vi "eDyno CAN Pack Signals.vi"(0 "Fault Injection":T5={"Imbalance ON"=FALSE, "Imbalance (g)"=0.5, "Misalignment ON"=FALSE, "Misalignment (g)"=0.2, "Bearing BPFO ON"=FALSE, "Bearing Impact (g)"=2.0, "Motor Ripple ON"=FALSE, "Torque Ripple (g)"=0.3, "PWM Noise ON"=FALSE, "PWM Level (g)"=0.05}, 5 "Speed Profile":T4={"Run-up Enabled"=FALSE, "Constant Speed (rpm)"=3000.0, "Run-up Start (rpm)"=500.0, "Run-up End (rpm)"=4500.0, "Run-up Duration (s)"=30.0}, 7 "Sim Config":T3={"Sample Rate (Hz)"=51200.0, "Ref Speed (rpm)"=3000.0, "Baseline 1x (g)"=0.02, "Noise Floor (g rms)"=0.01, "BPFO Order"=3.57, "Resonance (Hz)"=3500.0, "Decay (ms)"=0.8, "Pole Pairs"=4.0, "PWM Carrier (Hz)"=16000.0}, 9 "Fault Frequencies (Hz)":T2={"1x Shaft"=50.0, "2x Misalign"=100.0, "BPFO"=178.5, "Torque Ripple"=1200.0, "PWM Carrier"=16000.0}, 11 "Status":T1) -> (4 "Signal Values":dbl[](array[numeric]), 6 "Signal List":string[](array[string]), 8 "Active Fault Id":dbl)   [LabVIEW 2026]
doc: "PURPOSE\nConverts the eDyno simulator state into the 58 signal values of eDyno_NVH_PoC.dbc (v0.5) for an NI-XNET Signal Output Single-point session. Called once per CAN loop iteration.\n\nHOW TO USE\n1) Call it once before the loop and wire Signal List into XNET Create Session (Generic), mode Signal Output Single-point. Signal List is the single source of truth for the order of Signal Values.\n2) In the loop, wire Signal Values into XNET Write (Signal Single-point).\n\nINPUTS\n- Fault Injection, Speed Profile, Sim Config, Fault Frequencies (Hz): the simulator clusters, copied straight into the matching CAN signals.\n- Status: Speed Act (rpm) = shaft speed; Torque (Nm) = motor load torque (drives the MCU model); Block Counter = AO block index; Alive Counter = CAN loop iteration. Test Step and Seq State are no longer sent.\n\nDERIVED SIGNALS (one comment each on the block diagram)\n- Mode: 2 = run-up, 1 = constant speed.\n- AtSpeed: 1 when |Speed Act - target| < 1 rpm (target = Run-up End or Constant Speed).\n- ON flags: boolean -> 1/0.\n- ActiveId: 0 = none, 1..5 = the single fault that is on (Imbalance, Misalignment, BPFO, Torque ripple, PWM), 6 = more than one.\n- Alive counters: Alive Counter mod 16.\n- MCU_Status: computed by eDyno MCU Model.vi from speed and load torque.\n\nCHANGING THE DATABASE\nEvery DBC change must be mirrored here (signal list + values, same order). Check with src/CAN/_aixml/XNET Signal Probe.vi. FlexLogger 2026 Q3 does not decode DBCs with VAL_ value tables."
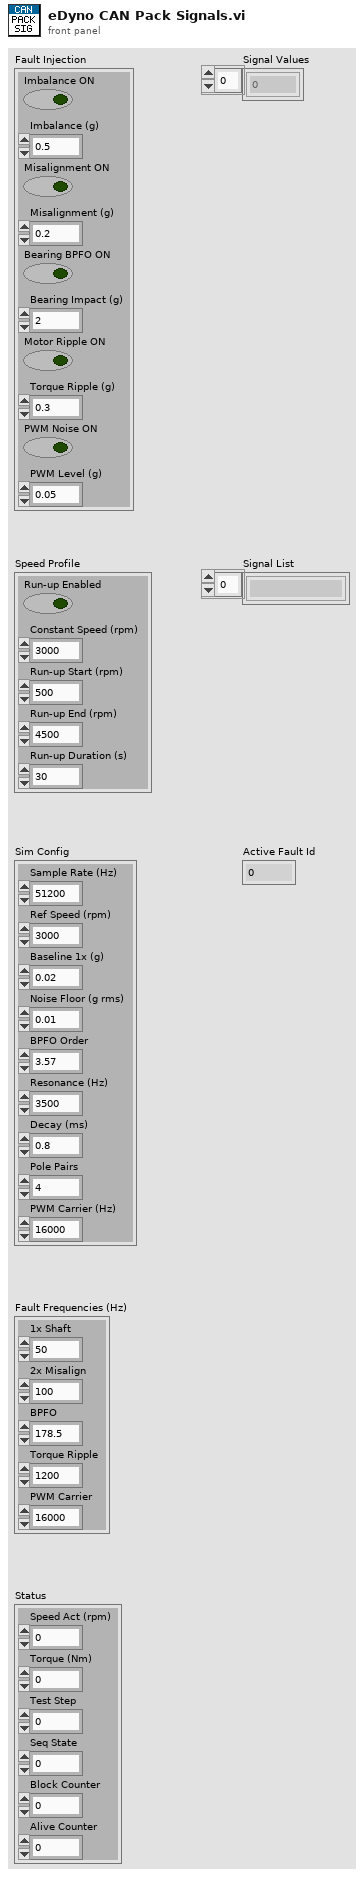
[diagram p1: front panel]
types:
  T1 = cluster{"Speed Act (rpm)":dbl, "Torque (Nm)":dbl, "Test Step":dbl, "Seq State":dbl, "Block Counter":dbl, "Alive Counter":dbl}
  T2 = cluster{"1x Shaft":dbl, "2x Misalign":dbl, "BPFO":dbl, "Torque Ripple":dbl, "PWM Carrier":dbl}
  T3 = cluster{"Sample Rate (Hz)":dbl, "Ref Speed (rpm)":dbl, "Baseline 1x (g)":dbl, "Noise Floor (g rms)":dbl, "BPFO Order":dbl, "Resonance (Hz)":dbl, "Decay (ms)":dbl, "Pole Pairs":dbl, "PWM Carrier (Hz)":dbl}
  T4 = cluster{"Run-up Enabled":bool, "Constant Speed (rpm)":dbl, "Run-up Start (rpm)":dbl, "Run-up End (rpm)":dbl, "Run-up Duration (s)":dbl}
  T5 = cluster{"Imbalance ON":bool, "Imbalance (g)":dbl, "Misalignment ON":bool, "Misalignment (g)":dbl, "Bearing BPFO ON":bool, "Bearing Impact (g)":dbl, "Motor Ripple ON":bool, "Torque Ripple (g)":dbl, "PWM Noise ON":bool, "PWM Level (g)":dbl}
  T6 = cluster{"Motor Speed (rpm)":dbl, "Torque (Nm)":dbl, "Phase Current RMS (A)":dbl, "DC Voltage (V)":dbl, "DC Current (A)":dbl, "Electrical Power (W)":dbl, "Winding Temp (degC)":dbl, "Controller Temp (degC)":dbl}
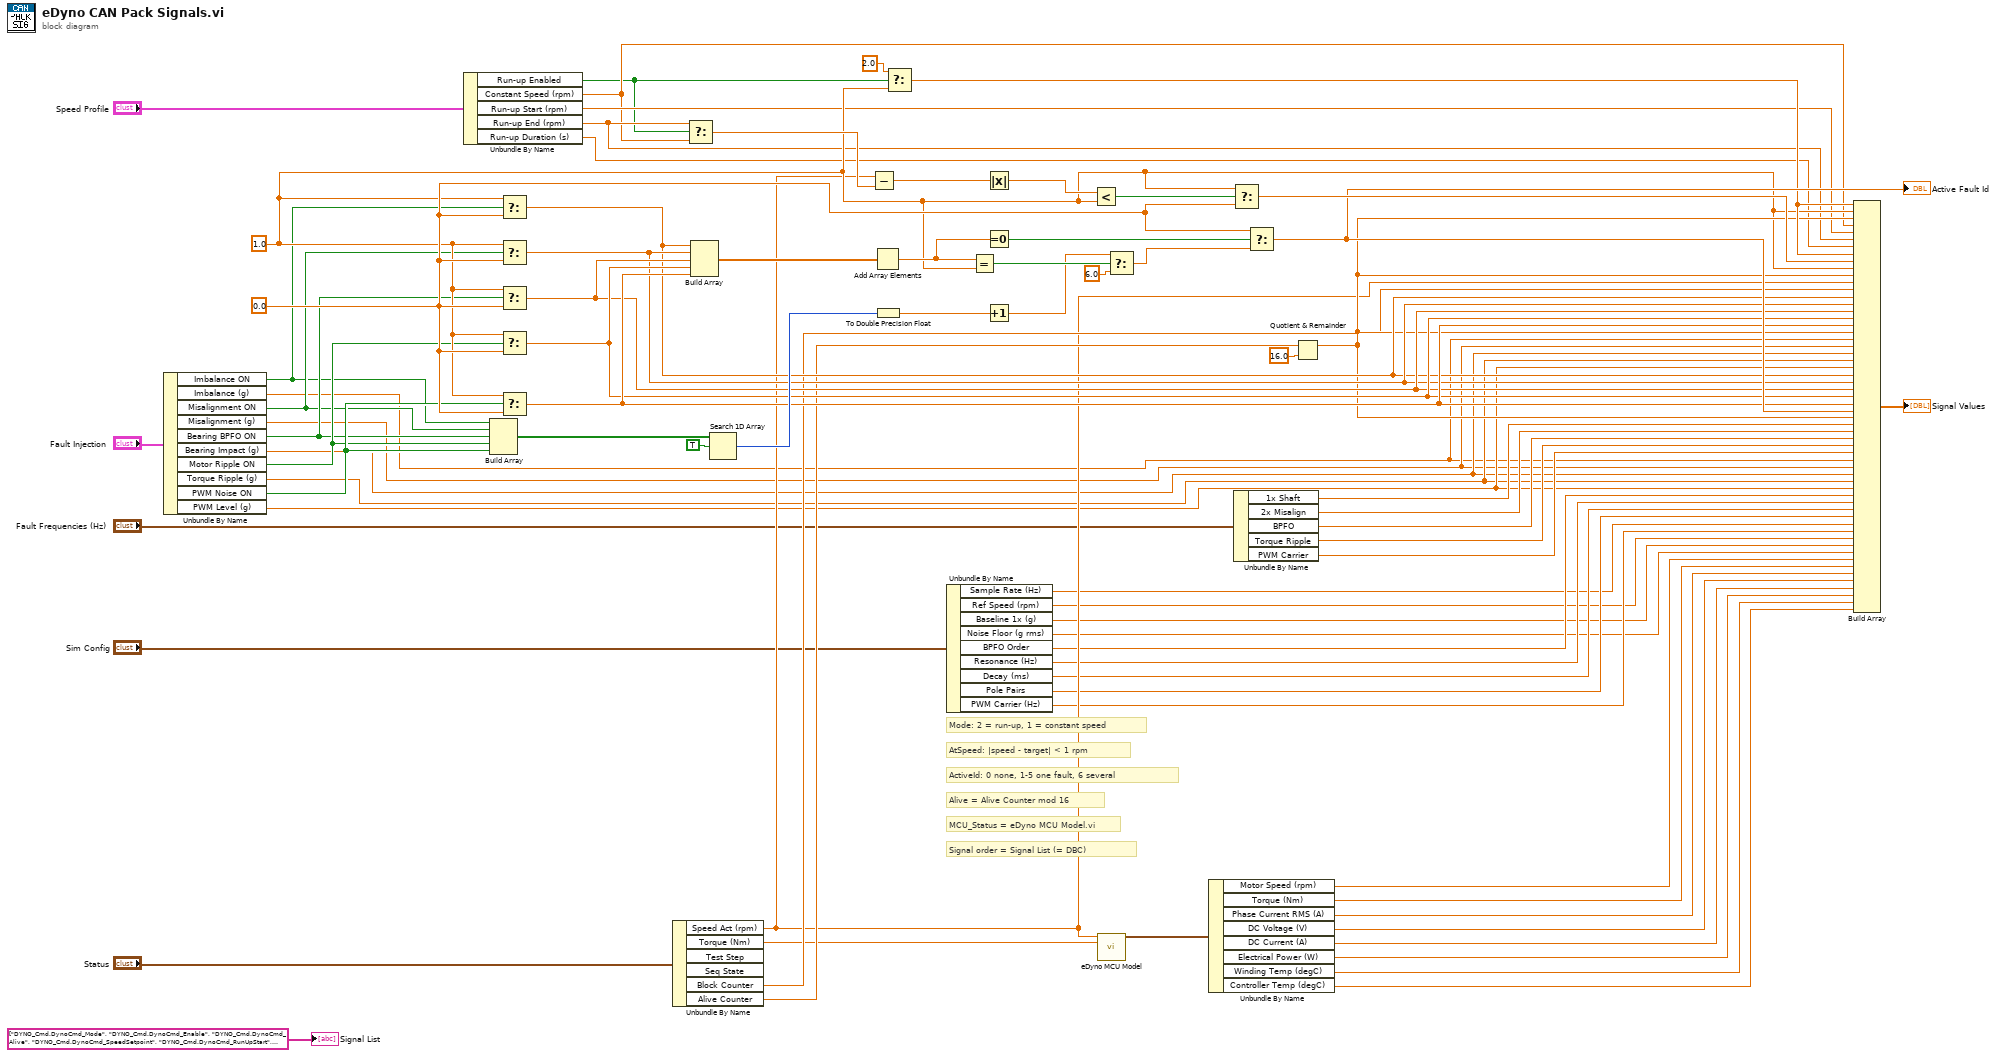
[diagram p0: block diagram]
diagram:
  w40 = 0.0 ("zero")
  w39 = 1.0 ("one")
  # "Signal order = Signal List (= DBC)"
  # "MCU_Status = eDyno MCU Model.vi"
  # "Alive = Alive Counter mod 16"
  # "ActiveId: 0 none, 1-5 one fault, 6 several"
  # "AtSpeed: |speed - target| < 1 rpm"
  # "Mode: 2 = run-up, 1 = constant speed"
  n1 = Unbundle By Name("Fault Injection") -> ("Imbalance ON"=w6:bool, "Imbalance (g)"=w7:dbl, "Misalignment ON"=w8:bool, "Misalignment (g)"=w9:dbl, "Bearing BPFO ON"=w10:bool, "Bearing Impact (g)"=w11:dbl, "Motor Ripple ON"=w12:bool, "Torque Ripple (g)"=w13:dbl, "PWM Noise ON"=w14:bool, "PWM Level (g)"=w15:dbl)
  n2 = Unbundle By Name("Speed Profile") -> ("Run-up Enabled"=w16:bool, "Constant Speed (rpm)"=w17:dbl, "Run-up Start (rpm)"=w18:dbl, "Run-up End (rpm)"=w19:dbl, "Run-up Duration (s)"=w20:dbl)
  n3 = Build Array(w6, w8, w10, w12, w14) -> (w55:bool[])
  n4 = Select(t=w39, s=w6, f=w40) -> (s? t:f=w50:dbl)
  n5 = Select(t=w39, s=w8, f=w40) -> (s? t:f=w51:dbl)
  n6 = Select(t=w39, s=w10, f=w40) -> (s? t:f=w52:dbl)
  n7 = Select(t=w39, s=w12, f=w40) -> (s? t:f=w53:dbl)
  n8 = Select(t=w39, s=w14, f=w40) -> (s? t:f=w54:dbl)
  n9 = Unbundle By Name("Status") -> ("Speed Act (rpm)"=w35:dbl, "Torque (Nm)"=w36:dbl, "Block Counter"=w37:dbl, "Alive Counter"=w38:dbl)  [unwired: 2 out]
  n10 = Select(t=w19, s=w16, f=w17) -> (s? t:f=w46:dbl)
  n11 = Build Array(w50, w51, w52, w53, w54) -> (w56:dbl[])
  n12 = Search 1D Array(1D array=w55, element=TRUE ("true")) -> (index of element=w59:i32)  [unwired: 1 in]
  n13 = Subtract(x=w35, y=w46) -> (x-y=w47:dbl)
  n14 = Add Array Elements(numeric array=w56) -> (sum=w57:dbl)
  n15 = To Double Precision Float(number=w59) -> (double precision float=w60:dbl)
  n16 = Select(t=2.0 ("two"), s=w16, f=w39) -> (s? t:f=w45:dbl)
  n17 = Unbundle By Name("Sim Config") -> ("Sample Rate (Hz)"=w21:dbl, "Ref Speed (rpm)"=w22:dbl, "Baseline 1x (g)"=w23:dbl, "Noise Floor (g rms)"=w24:dbl, "BPFO Order"=w25:dbl, "Resonance (Hz)"=w26:dbl, "Decay (ms)"=w27:dbl, "Pole Pairs"=w28:dbl, "PWM Carrier (Hz)"=w29:dbl)
  n18 = Equal?(x=w57, y=w39) -> (x = y?=w62:bool)
  n19 = Absolute Value(x=w47) -> (abs(x)=w48:dbl)
  n20 = Equal To 0?(x=w57) -> (x = 0?=w63:bool)
  n21 = Increment(x=w60) -> (x+1=w61:dbl)
  n22 = Less?(x=w48, y=w39) -> (x < y?=w49:bool)
  n23 = call "eDyno MCU Model.vi"("Speed (rpm)"=w35, "Load Torque (Nm)"=w36) -> ("MCU Status"=w67:T6)  [unwired: 13 in]
  n24 = Select(t=w61, s=w62, f=6.0 ("six")) -> (s? t:f=w64:dbl)
  n25 = Unbundle By Name(w67) -> ("Motor Speed (rpm)"=w68:dbl, "Torque (Nm)"=w69:dbl, "Phase Current RMS (A)"=w70:dbl, "DC Voltage (V)"=w71:dbl, "DC Current (A)"=w72:dbl, "Electrical Power (W)"=w73:dbl, "Winding Temp (degC)"=w74:dbl, "Controller Temp (degC)"=w75:dbl)
  n26 = Select(t=w39, s=w49, f=w40) -> (s? t:f=w66:dbl)
  n27 = Unbundle By Name("Fault Frequencies (Hz)") -> ("1x Shaft"=w30:dbl, "2x Misalign"=w31:dbl, "BPFO"=w32:dbl, "Torque Ripple"=w33:dbl, "PWM Carrier"=w34:dbl)
  n28 = Select(t=w40, s=w63, f=w64) -> (s? t:f=w65:dbl)
  "Active Fault Id" <- w65
  n29 = Quotient & Remainder(x=w38, y=16.0 ("sixteen")) -> (x-y*floor(x/y)=w44:dbl)  [unwired: 1 out]
  n30 = Build Array(w45, w39, w44, w17, w18, w19, w20, w45, w66, w39, w44, w35, w37, w50, w51, w52, w53, w54, w44, w7, w9, w11, w13, w15, w50, w51, w52, w53, w54, w65, w44, w30, w31, w32, w33, w34, w7, w9, w11, w13, w15, w25, w26, w27, w28, w21, w29, w22, w23, w24, w68, w69, w70, w71, w72, w73, w74, w75) -> (→"Signal Values":dbl[])
  "Signal List" <- string[] ["DYNO_Cmd.DynoCmd_Mode", "DYNO_Cmd.DynoCmd_Enable", "DYNO_Cmd.DynoCmd_Alive", "DYNO_Cmd.DynoCmd_SpeedSetpoint", "DYNO_Cmd.DynoCmd_RunUpStart", "DYNO_Cmd.DynoCmd_RunUpEnd", "DYNO_Cmd.DynoCmd_RunUpDuration", "DYNO_Status.DynoSts_Mode", "DYNO_Status.DynoSts_AtSpeed", "DYNO_Status.DynoSts_SimRunning", "DYNO_Status.DynoSts_Alive", "DYNO_Status.DynoSts_SpeedAct", "DYNO_Status.DynoSts_BlockCounter", "SIM_FaultCmd.FltCmd_Imbalance_On", "SIM_FaultCmd.FltCmd_Misalign_On", "SIM_FaultCmd.FltCmd_BPFO_On", "SIM_FaultCmd.FltCmd_Ripple_On", "SIM_FaultCmd.FltCmd_PWM_On", "SIM_FaultCmd.FltCmd_Alive", "SIM_FaultCmd.FltCmd_Imbalance_Amp", "SIM_FaultCmd.FltCmd_Misalign_Amp", "SIM_FaultCmd.FltCmd_BPFO_Amp", "SIM_FaultCmd.FltCmd_Ripple_Amp", "SIM_FaultCmd.FltCmd_PWM_Amp", "SIM_FaultStatus.FltSts_Imbalance_On", "SIM_FaultStatus.FltSts_Misalign_On", "SIM_FaultStatus.FltSts_BPFO_On", "SIM_FaultStatus.FltSts_Ripple_On", "SIM_FaultStatus.FltSts_PWM_On", "SIM_FaultStatus.FltSts_ActiveId", "SIM_FaultStatus.FltSts_Alive", "SIM_FaultStatus.FltSts_Freq_1x", "SIM_FaultStatus.FltSts_Freq_2x", "SIM_FaultStatus.FltSts_Freq_BPFO", "SIM_FaultStatus.FltSts_Freq_Ripple", "SIM_FaultStatus.FltSts_Freq_PWM", "SIM_FaultStatus.FltSts_Imbalance_Amp", "SIM_FaultStatus.FltSts_Misalign_Amp", "SIM_FaultStatus.FltSts_BPFO_Amp", "SIM_FaultStatus.FltSts_Ripple_Amp", "SIM_FaultStatus.FltSts_PWM_Amp", "SIM_Config.SimCfg_BPFO_Order", "SIM_Config.SimCfg_Resonance", "SIM_Config.SimCfg_Decay", "SIM_Config.SimCfg_PolePairs", "SIM_Config.SimCfg_SampleRate", "SIM_Config.SimCfg_PWMCarrier", "SIM_Config.SimCfg_RefSpeed", "SIM_Config.SimCfg_Baseline1x", "SIM_Config.SimCfg_NoiseFloor", "MCU_Status.MCU_MotorSpeed", "MCU_Status.MCU_TorqueEst", "MCU_Status.MCU_PhaseCurrentRms", "MCU_Status.MCU_DCVoltage", "MCU_Status.MCU_DCCurrent", "MCU_Status.MCU_ElecPower", "MCU_Status.MCU_WindingTemp", "MCU_Status.MCU_ControllerTemp"] ("signal list")
